vi "Update UI Details.vi"(8 "error in":errorcluster, 9 "UI path":path, 10 "measurement service name":string, 11 "project ref":refnum<vi>) -> (0 "error out":errorcluster, 3 "project ref out":refnum<vi>)   [LabVIEW 2021, in "MeasurementService Editor.lvlib"]
uses:
  MeasurementService Editor.lvlib
  <vilib>/Plug-In SDKs/Measurements/Helpers/TypeDefs/User Interface Information.ctl
  <vilib>/Plug-In SDKs/Measurements/NI Measurement Plug-In SDK.lvlib
  Converter/Converter Reusables/Converter Reusables.lvlib
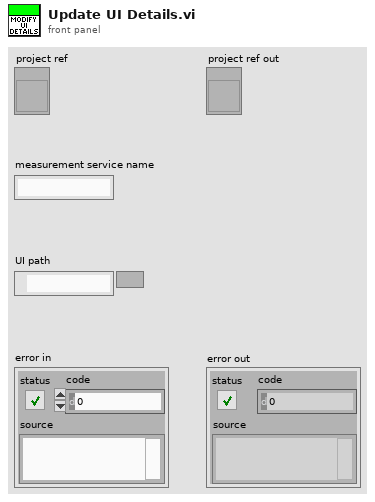
[diagram p1: front panel]
types:
  T1 = typedef "NI Measurement Plug-In SDK.lvlib/User Interface Information.ctl" = cluster{"file":string}
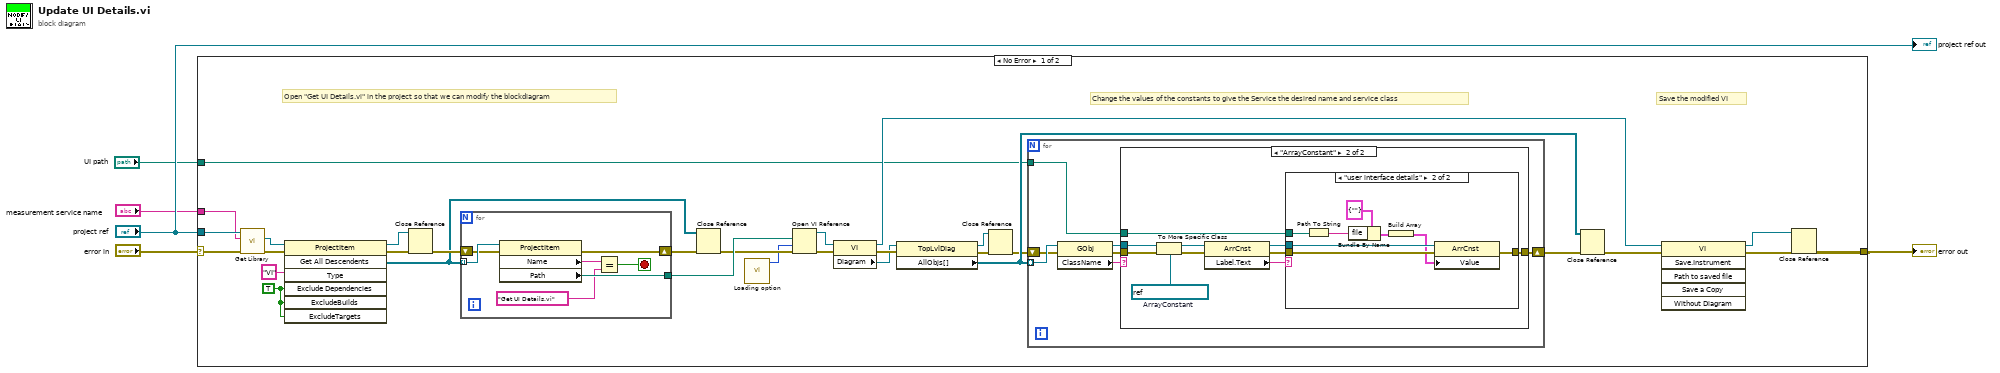
[diagram p0: block diagram]
diagram:
  n1 = case shown="No Error" "error in" {
    selector: "error in" -> [w23 w70]
    tunnel: "project ref" -> [w22 _]
    tunnel: [w33 w70] -> w3
    tunnel: "measurement service name" -> [w16 _]
    tunnel: "UI path" -> [w9 _]
    frame No Error {
      w35 = TRUE ("ExcludeDependencies")
      # "Save the modified VI"
      # "Open \"Get UI Details.vi\" in the project so that we can modify the blockdiagram"
      # "Change the values of the constants to give the Service the desired name and service class"
      n2 = call "Get Library.vi"("error in (no error)"=w23, "library name"=w16, "project ref"=w22) -> ("error out"=w21:errorcluster, "library item"=w20:refnum<vi>)  [unwired: 5 in, 2 out]
      n3 = invoke class="ProjectItem" method="Get All Descendents"(reference=w20, error in=w21, "Type"="VI", "Exclude Dependencies"=w35, "ExcludeBuilds"=w35, "ExcludeTargets"=w35) -> (reference out=w17:refnum<vi>, error out=w19:errorcluster, "All Descendents"=w7:refnum<vi>[])  [unwired: 1 in, 4 out]
      n4 = Close Reference(reference=w17, error in (no error)=w19) -> (error out=w18:errorcluster)
      n5 = for {
        tunnel: w7 -> [w69] mode=indexing
        shift-right: [w64] -> w14
        shift-left: w18 -> [w67]
        tunnel: [w65] -> w15
        stop <- w66 stop-if-true
        n6 = property class="ProjectItem"(reference=w69, error in=w67) -> (error out=w64:errorcluster, "Name"=w68:string, "Path"=w65:path)  [unwired: 1 out]
        n7 = Equal?(x=w68, y="Get UI Details.vi") -> (x = y?=w66:bool)
      }
      n8 = Close Reference(reference=w7, error in (no error)=w14) -> (error out=w8:errorcluster)
      n9 = call "Loading option.vi"() -> ("options"=w6:i32)  [unwired: 11 in]
      n10 = Open VI Reference(vi path=w15, options=w6, error in (no error)=w8) -> (vi reference=w30:refnum<vi>, error out=w28:errorcluster)  [unwired: 3 in]
      n11 = property class="VI"(reference=w30, error in=w28) -> (reference out=w26:refnum<vi>, error out=w29:errorcluster, "Diagram"=w27:refnum<vi>)
      n12 = property class="TopLvlDiag"(reference=w27, error in=w29) -> (reference out=w10:refnum<vi>, error out=w12:errorcluster, "AllObjs[]"=w13:refnum<vi>[])
      n13 = Close Reference(reference=w10, error in (no error)=w12) -> (error out=w11:errorcluster)
      n14 = for {
        tunnel: w13 -> [w42] mode=indexing
        shift-right: [w38] -> w25
        shift-left: w11 -> [w41]
        tunnel: w9 -> [w36]
        n15 = property class="GObj"(reference=w42, error in=w41) -> (reference out=w40:refnum<vi>, error out=w39:errorcluster, "ClassName"=w37:string)
        n16 = case shown="\"ArrayConstant\"" w37 {
          tunnel: w40 -> [_ w52]
          tunnel: w39 -> [w43 w51]
          tunnel: w36 -> [_ w50]
          tunnel: [w43 w49] -> w38
          frame Default {
          }
          frame "ArrayConstant" {
            w53 = refnum<vi> refnum  # ArrayConstant
            n17 = To More Specific Class(target class=w53, reference=w52, error in=w51) -> (specific class reference=w48:refnum<vi>, error out=w47:errorcluster)
            n18 = property class="ArrCnst"(reference=w48, error in=w47) -> (reference out=w46:refnum<vi>, error out=w45:errorcluster, "Label.Text"=w44:string)
            n19 = case shown="\"user interface details\"" w44 {
              tunnel: w50 -> [_ w56]
              tunnel: [w54 w62] -> w49
              tunnel: w46 -> [_ w61]
              tunnel: w45 -> [w54 w60]
              frame Default {
              }
              frame "user interface details" {
                n20 = Path To String(path=w56) -> (string=w55:string)
                n21 = Bundle By Name(cluster=T1 {"file"=""} ("UI Information"), "file"=w55) -> (w58:T1)
                n22 = Build Array(w58) -> (w57:T1[])
                n23 = property class="ArrCnst"(reference=w61, error in=w60, "Value"=w57) -> (error out=w62:errorcluster)  [unwired: 1 out]
              }
            }
          }
        }
      }
      n24 = Close Reference(reference=w13, error in (no error)=w25) -> (error out=w24:errorcluster)
      n25 = invoke class="VI" method="Save.Instrument"(reference=w26, error in=w24) -> (reference out=w32:refnum<vi>, error out=w31:errorcluster)  [unwired: 4 in, 4 out]
      n26 = Close Reference(reference=w32, error in (no error)=w31) -> (error out=w33:errorcluster)
    }
    frame Error {
    }
  }
  "error out" <- w3
  "project ref out" <- "project ref"
